vi "SPI Write&Read.vi"(8 "error in (no error)":errorcluster, 10 "Data to Write":u8[](array[numeric]), 11 "SPI Device":T1) -> (0 "error out":errorcluster, 2 "Data readed":u8[](array[numeric]) format="%0d", 3 "SPI Device out":T1)   [LabVIEW 2020, in "wiringPi.lvlib"]
doc: "<b>_______________________________________________________________</b>\n** Author: Juan José Villacorta\n** LabVIEW wrapper for C library <b> wiringPi </b>,\n** https://github.com/WiringPi/WiringPi\n<b>_______________________________________________________________</b>\n/*\n * Write and Read data to/from a SPI Device\n * On SPI the data transfers are duplex, so the size of the data readed is the same \n * of the data writen\n**********************************************************************************\n*/"
uses:
  wiringPi.lvlib
  Type Defs/SPI Dev.ctl
  Type Defs/SPI Channel.ctl
  Type Defs/SPI Device.ctl
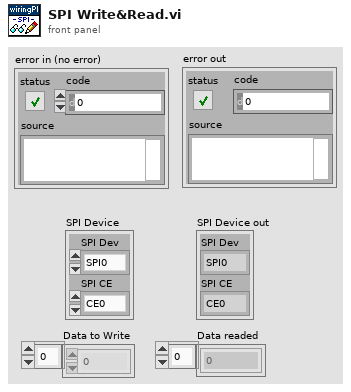
[diagram p1: front panel]
types:
  T1 = typedef "wiringPi.lvlib/SPI Device.ctl" = cluster{"SPI Dev":T2, "SPI CE":T3}
  T2 = typedef "wiringPi.lvlib/SPI Dev.ctl" = enum32{"SPI0", "SPI1"}
  T3 = typedef "wiringPi.lvlib/SPI Channel.ctl" = enum32{"CE0", "CE1", "CE2"}
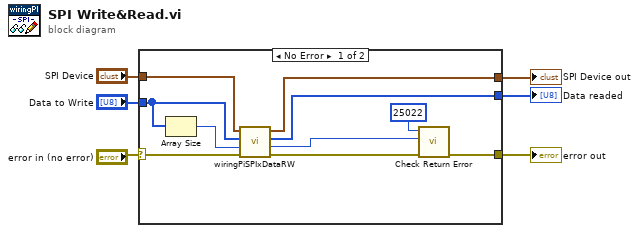
[diagram p0: block diagram]
diagram:
  n1 = case shown="No Error" "error in (no error)" {
    selector: "error in (no error)" -> [w15 w17]
    tunnel: [w10 w17] -> w5
    tunnel: "Data to Write" -> [w14 _]
    tunnel: [w11 _] -> w3
    tunnel: "SPI Device" -> [w13 w18]
    tunnel: [w12 w18] -> w1
    frame No Error {
      n2 = Array Size(array=w14) -> (size(s)=w16:i32)
      n3 = call "wiringPiSPIxDataRW.vi"("error in (no error)"=w15, "len"=w16, "data in"=w14, "SPI Device"=w13) -> ("error out"=w8:errorcluster, "return"=w9:i32, "data out"=w11:u8[], "SPI Device out"=w12:T1)  [unwired: 4 in]
      n4 = call "Check Return Error.vi"("error in (no error)"=w8, "Return code"=w9, "Error number"=25022) -> ("error out"=w10:errorcluster)  [unwired: 8 in]
    }
    frame Error {
    }
  }
  "error out" <- w5
  "Data readed" <- w3
  "SPI Device out" <- w1
